vi "new report subVI.vi"(0 "report in":refnum<class "ooWriter.lvclass">, 1 "window state (normal)":T1(ring)=enum."normal", 5 "display alerts? (F)":bool, 7 "template (empty)":path, 9 "machine name (empty)":string, 11 "error in (no error)":errorcluster) -> (4 "report out":refnum<class "ooWriter.lvclass">, 15 "error out":errorcluster)   [LabVIEW 2009, in "ooWriter.lvclass"]
uses:
  ooWriter.lvclass
  ooDocument/ooDocument.lvclass
  C:/Projets/LAVAG/OpenOfficeRGT/AODL/DLLs/AODL.dll
  ooWriter.lvclass/ooWriter.ctl
  <vilib>/Utility/NIReport.llb/NI_ReportGenerationCore.lvlib
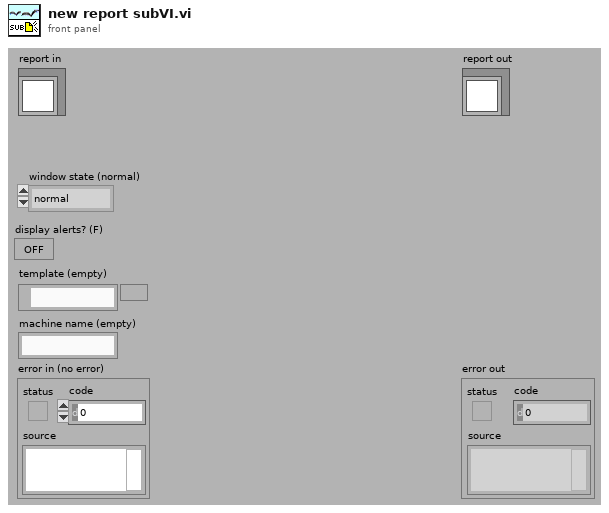
[diagram p1: front panel]
types:
  T1 = enum16{"maximized", "minimized", "normal", "no change"}
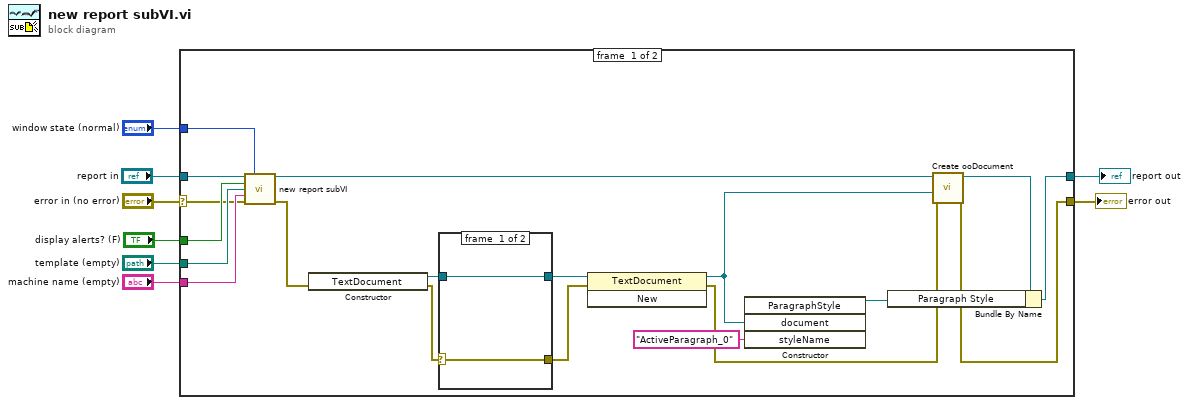
[diagram p0: block diagram]
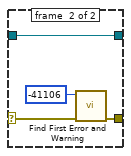
[diagram p2: hidden frame]
diagram:
  n1 = case shown="No Error" "error in (no error)" {
    selector: "error in (no error)" -> [w22 w34]
    tunnel: "report in" -> [w27 w35]
    tunnel: "window state (normal)" -> [w26 _]
    tunnel: [w21 w35] -> w6
    tunnel: "template (empty)" -> [w25 _]
    tunnel: "machine name (empty)" -> [w24 _]
    tunnel: [w10 w34] -> w3
    tunnel: "display alerts? (F)" -> [w23 _]
    frame #0 {
      n2 = call-parent "new report subVI.vi"("report in"=w27, "window state (normal)"=w26, "display alerts? (F)"=w23, "template (empty)"=w25, "machine name (empty)"=w24, "error in (no error)"=w22) -> ("report out"=w14:refnum<class "ooWriter.lvclass">, "error out"=w20:errorcluster)  [unwired: 8 in]
      n3 = constructor class="TextDocument"(error in=w20) -> (reference out=w18:refnum<k24>, error out=w19:errorcluster)  [unwired: 2 in, 1 out]
      n4 = case shown="Error" w19 {
        selector: w19 -> [w29 w31]
        tunnel: [w29 w32] -> w16
        tunnel: [w28 w30] -> w17
        tunnel: w18 -> [w28 w30]
        frame #0 {
        }
        frame #1 {
          n5 = call <vilib>:"Find First Error and Warning.vi"("error in (no error)"=w31, "error code"=-41106) -> ("error out"=w32:errorcluster)  [unwired: 5 out]
        }
      }
      n6 = invoke class="TextDocument" method="New"(reference=w17, error in=w16) -> (reference out=w12:refnum<k24>, error out=w11:errorcluster)  [unwired: 1 in, 1 out]
      n7 = constructor class="ParagraphStyle"("document"=w12, "styleName"="ActiveParagraph_0") -> (reference out=w9:refnum<k24>)  [unwired: 3 in, 4 out]
      n8 = call-dynamic "Create ooDocument.vi"("error in (no error)"=w11, "Document"=w12, "ooDocument in"=w14) -> ("error out"=w10:errorcluster, "ooDocument out"=w13:refnum<class "ooWriter.lvclass">)  [unwired: 7 in]
      n9 = Bundle By Name(cluster=w13, "Paragraph Style"=w9) -> (w21:refnum<class "ooWriter.lvclass">)
    }
    frame #1 {
    }
  }
  "error out" <- w3
  "report out" <- w6
